vi "Get Node.vi"(8 "error in (no error)":errorcluster, 10 "Node":string, 11 "Test Result in":refnum<class "Test Result.lvclass">) -> (0 "error out":errorcluster, 1 "Assertions":T3[](array[typedef]), 2 "Test Node":T1, 3 "Test Result out":refnum<class "Test Result.lvclass">, 4 "found":bool, 5 "indent level":i32)   [LabVIEW 2020, in "Caraya.lvlib" / "Test Result.lvclass"]
uses:
  Test Result.lvclass
  Assert Event Data.ctl
  Test Node.ctl
  Test Registration Data.ctl
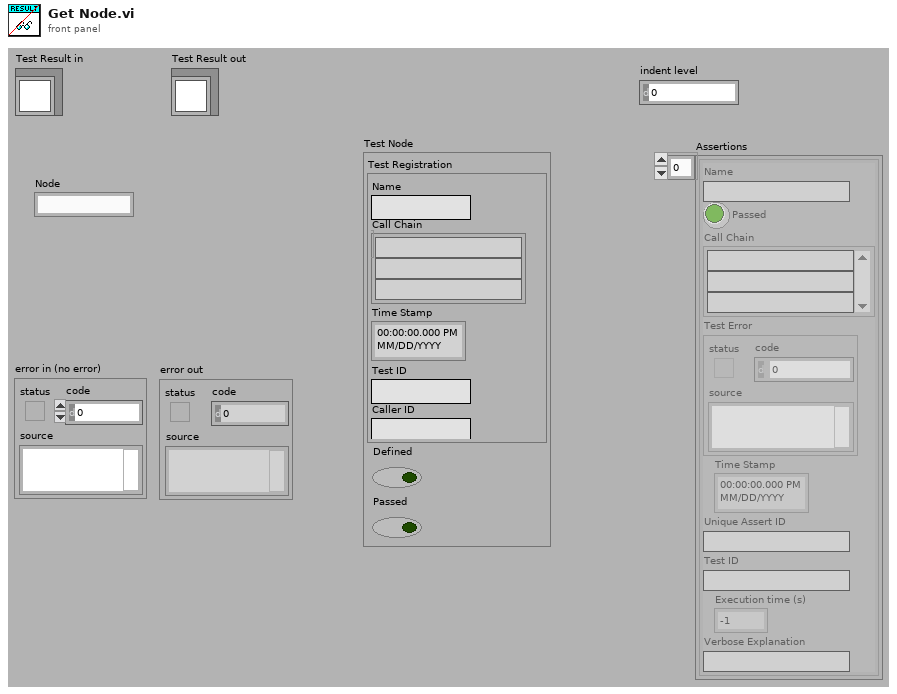
[diagram p1: front panel]
types:
  T1 = typedef "Caraya.lvlib/Test Result.lvclass/Test Node.ctl" = cluster{"Test Registration":T2, "Defined":bool, "Passed":bool}
  T2 = typedef "Caraya.lvlib/Test Result.lvclass/Test Registration Data.ctl" = cluster{"Name":string, "Call Chain":string[], "Time Stamp":timestamp, "Test ID":string, "Caller ID":string}
  T3 = typedef "Caraya.lvlib/Test Result.lvclass/Assert Event Data.ctl" = cluster{"Name":string, "Passed":bool, "Call Chain":string[], "Test Error":errorcluster, "Time Stamp":timestamp, "Unique Assert ID":string, "Test ID":string, "Execution time (s)":dbl, "Verbose Explanation":string}
  T4 = typedef "Caraya.lvlib/Test Result.lvclass/Assert Event Data (Extended).ctl" = cluster{"name":string, "passed":bool, "call-chain":string[], "test-error":errorcluster, "timestamp":timestamp, "assert-id":string, "test-id":string, "time":dbl, "message":string, "properties":variant, "measurements":variant, "user-defined":variant}
  T5 = typedef "Caraya.lvlib/Test Result.lvclass/Test Node (Extended).ctl" = cluster{"Test Registration":T2, "Defined":bool, "Passed":bool, "properties":variant}
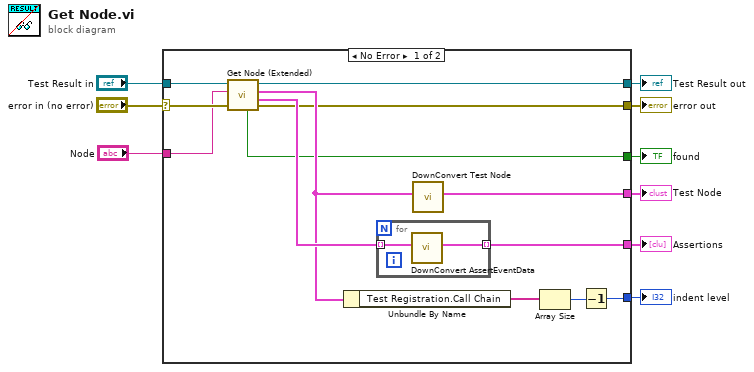
[diagram p0: block diagram]
diagram:
  n1 = case shown="No Error" "error in (no error)" {
    selector: "error in (no error)" -> [w11 w26]
    tunnel: [w12 w26] -> w8
    tunnel: [w14 w25] -> w6
    tunnel: "Test Result in" -> [w17 w25]
    tunnel: "Node" -> [w10 _]
    tunnel: [w13 _] -> w4
    tunnel: [w18 _] -> w2
    tunnel: [w19 _] -> w3
    tunnel: [w20 _] -> w1
    frame No Error {
      n2 = call "Get Node (Extended).vi"("error in (no error)"=w11, "Node"=w10, "Test Result in"=w17) -> ("error out"=w12:errorcluster, "Assertions"=w16:T4[], "Test Node"=w15:T5, "Test Result out"=w14:refnum<class "Test Result.lvclass">, "found"=w13:bool)  [unwired: 3 in, 1 out]
      n3 = Unbundle By Name(w15) -> ("Test Registration.Call Chain"=w22:string[])
      n4 = for {
        tunnel: w16 -> [w24] mode=indexing
        tunnel: [w23] -> w19 mode=indexing
        n5 = call "DownConvert AssertEventData.vi"("Assert Event Data (Extended)"=w24) -> ("Assert Event Data"=w23:T3)  [unwired: 10 in]
      }
      n6 = call "DownConvert Test Node.vi"("Test Node (Extended)"=w15) -> ("Test Node"=w18:T1)  [unwired: 10 in]
      n7 = Array Size(array=w22) -> (size(s)=w21:i32)
      n8 = Decrement(x=w21) -> (x-1=w20:i32)
    }
    frame Error {
    }
  }
  "error out" <- w8
  "Test Result out" <- w6
  "found" <- w4
  "Assertions" <- w3
  "Test Node" <- w2
  "indent level" <- w1
